vi "GetTestTypeDescv1NoRbac.vi"() -> ()   [LabVIEW 2017]
uses:
  <userlib>/_RADE/japc/classes/JGet/JGet.lvclass
  <vilib>/Analysis/NI_AALBase.lvlib
panel:
  out "standard deviation":dbl format="%0.2f"
  out "test_property":T1
  out "mean":dbl format="%0.2f"
  out "error out":errorcluster
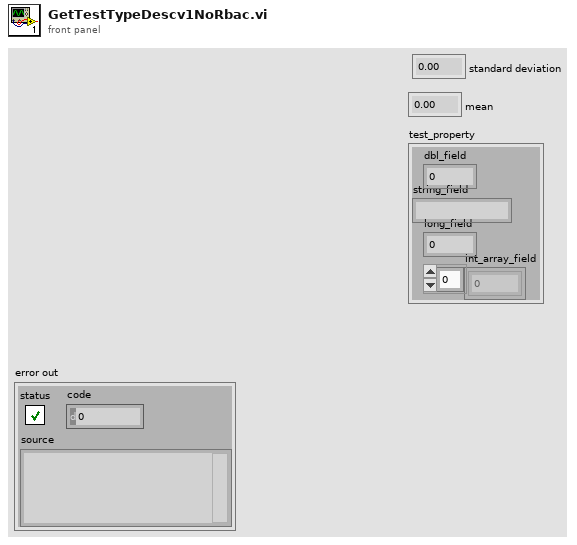
[diagram p1: front panel]
types:
  T1 = cluster{"dbl_field":dbl, "string_field":string, "long_field":i64, "int_array_field":i32[]}
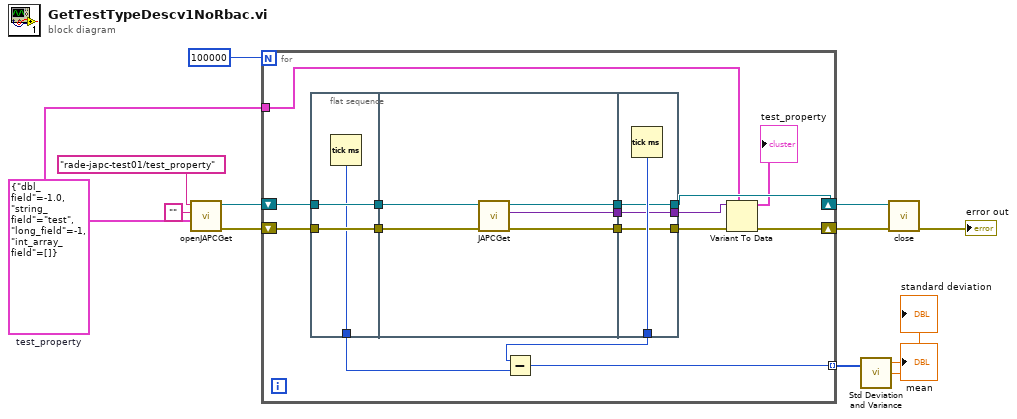
[diagram p0: block diagram]
diagram:
  w3 = T1 {"dbl_field"=-1.0, "string_field"="test", "long_field"=-1, "int_array_field"=[]}  # test_property
  n1 = call <userlib>:"openJAPCGet.vi"("Data type"=w3, "Cycle"="", "URL"="rade-japc-test01/test_property") -> ("error out"=w8:errorcluster, "Object out"=w9:refnum<class "JGet.lvclass">)  [unwired: 7 in]
  n2 = for {
    N: 100000 -> [_]
    tunnel: [w24] -> w6 mode=indexing
    shift-right: [w18] -> w4
    shift-left: w8 -> [w25]
    shift-right: [w17] -> w2
    shift-left: w9 -> [w27]
    tunnel: w3 -> [w16]
    n3 = flat-sequence {
      tunnel: [w31] -> w28
      tunnel: w27 -> [w31]
      tunnel: [w30] -> w26
      tunnel: w25 -> [w30]
      tunnel: [w29] -> w23
      tunnel: w28 -> [w36]
      tunnel: w26 -> [w35]
      tunnel: [w34] -> w21
      tunnel: [w33] -> w20
      tunnel: [w32] -> w14
      tunnel: [w40] -> w22
      tunnel: [w39] -> w17
      tunnel: w21 -> [w39]
      tunnel: [w38] -> w19
      tunnel: w20 -> [w38]
      tunnel: [w37] -> w13
      tunnel: w14 -> [w37]
      frame #0 {
        n4 = Tick Count (ms)() -> (millisecond timer value=w29:u32)
      }
      frame #1 {
        n5 = call <userlib>:"JAPCGet.vi"("error in (no error)"=w35, "Object in"=w36) -> ("error out"=w33:errorcluster, "Data"=w32:variant, "Object out"=w34:refnum<class "JGet.lvclass">)  [unwired: 5 in, 2 out]
      }
      frame #2 {
        n6 = Tick Count (ms)() -> (millisecond timer value=w40:u32)
      }
    }
    n7 = Subtract(x=w22, y=w23) -> (x-y=w24:u32)
    n8 = Variant To Data(error in=w19, type=w16, Variant=w13) -> (data=→"test_property":T1, error out=w18:errorcluster)
  }
  n9 = call <vilib>:"Std Deviation and Variance.vi"("X"=w6) -> ("mean"=→"mean":dbl, "standard deviation"=→"standard deviation":dbl)  [unwired: 1 in, 1 out]
  n10 = call-dynamic "close.vi"("error in (no error)"=w4, "Object in"=w2) -> ("error out"=→"error out":errorcluster)  [unwired: 9 in]
